vi "Convert Ultras. sensor V to L-min.vi"(11 "Waveform":dbl) -> (3 "Numeric":dbl)   [LabVIEW 2024]
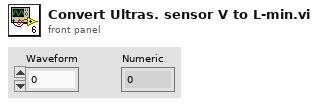
[diagram p1: front panel]
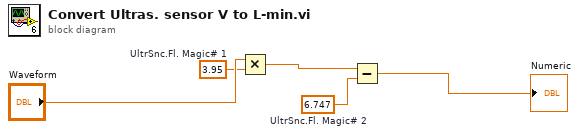
[diagram p0: block diagram]
diagram:
  w3 = 6.747  # UltrSnc.Fl. Magic# 2
  w4 = 3.95  # UltrSnc.Fl. Magic# 1
  n1 = Multiply(x="Waveform", y=w4) -> (x*y=w2:dbl)
  n2 = Subtract(x=w2, y=w3) -> (x-y=→"Numeric":dbl)
